vi "InitUI.vi"(8 "error in":errorcluster, 9 "Data":cluster{"UITitle":string, "HideUI":bool}, 11 "UI_Library in":refnum<class "UI_Library.lvclass">) -> (0 "error out":errorcluster, 3 "UI_Library out":refnum<class "UI_Library.lvclass">)   [LabVIEW 2018, in "UI_Library.lvlib" / "UI_Library.lvclass"]
uses:
  UI_Library.lvclass
  UI_Library.lvclass/UI_Library.ctl
  <vilib>/Utility/miscctls.llb/LVPointTypeDef.ctl
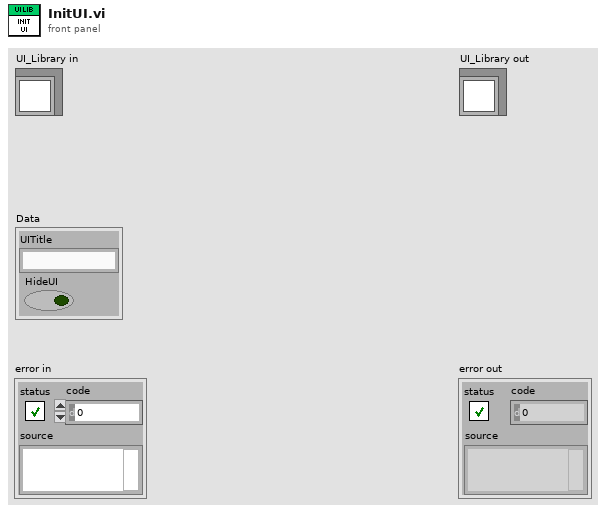
[diagram p1: front panel]
types:
  T1 = enum32{"Invalid", "Standard", "Closed", "Hidden", "Minimized", "Maximized"}
  T2 = typedef "LVPointTypeDef.ctl" = cluster{"Horizontal":i16, "Vertical":i16}
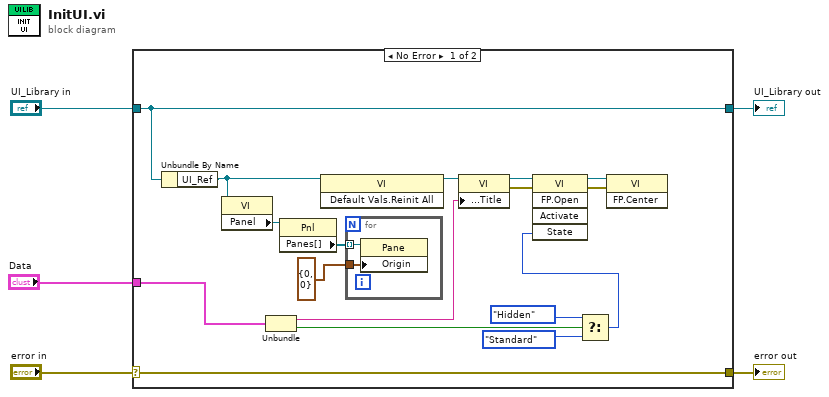
[diagram p0: block diagram]
diagram:
  n1 = case shown="No Error" "error in" {
    selector: "error in" -> [w22 w26]
    tunnel: [w22 w26] -> w4
    tunnel: [w8 w25] -> w2
    tunnel: "UI_Library in" -> [w8 w25]
    tunnel: "Data" -> [w6 _]
    frame No Error {
      n2 = Unbundle By Name(w8) -> ("UI_Ref"=w7:refnum<vi>)
      n3 = property on="Property Node" class="VI"(reference=w7) -> ("Panel"=w13:refnum<vi>)  [unwired: 1 in, 2 out]
      n4 = Unbundle(w6) -> ("UITitle"=w9:string, "HideUI"=w10:bool)
      n5 = property on="Property Node" class="Pnl"(reference=w13) -> ("Panes[]"=w12:refnum<vi>[])  [unwired: 1 in, 2 out]
      n6 = invoke class="VI" method="Default Vals.Reinit All"(reference=w7) -> (reference out=w14:refnum<vi>)  [unwired: 2 in, 2 out]
      n7 = for {
        tunnel: w12 -> [w24] mode=indexing
        tunnel: T2 {"Horizontal"=0, "Vertical"=0} ("Origin") -> [w23]
        n8 = property on="Property Node" class="Pane"(reference=w24, "Origin"=w23) -> ()  [unwired: 1 in, 2 out]
      }
      n9 = property on="Property Node" class="VI"(reference=w14, "Front Panel.Title"=w9) -> (reference out=w19:refnum<vi>, error out=w21:errorcluster)  [unwired: 1 in]
      n10 = Select(t=T1."Hidden" ("State"), s=w10, f=T1."Standard" ("State")) -> (s? t:f=w15:T1)
      n11 = invoke on="Invoke Node" class="VI" method="FP.Open"(reference=w19, error in=w21, "State"=w15) -> (reference out=w18:refnum<vi>, error out=w20:errorcluster)  [unwired: 2 in, 3 out]
      n12 = invoke on="Invoke Node" class="VI" method="FP.Center"(reference=w18, error in=w20) -> ()  [unwired: 1 in, 3 out]
    }
    frame Error {
    }
  }
  "error out" <- w4
  "UI_Library out" <- w2
